vi "Histogram Plot save.vi"(6 "R Con H":dbl[][](array[numeric]), 7 "Date":string, 8 "error in":errorcluster caption="エラー入力", 9 "Normalized Plot Graph":dbl[][](graph), 10 "Plot Graph":dbl[][](graph), 11 "Folder Path":string) -> (0 "error out":errorcluster caption="エラー出力")   [LabVIEW 2018]
panel:
  out "Normalized Histogram":dbl[][](array[numeric])
  out "Count Historam":i32[][](array[numeric])
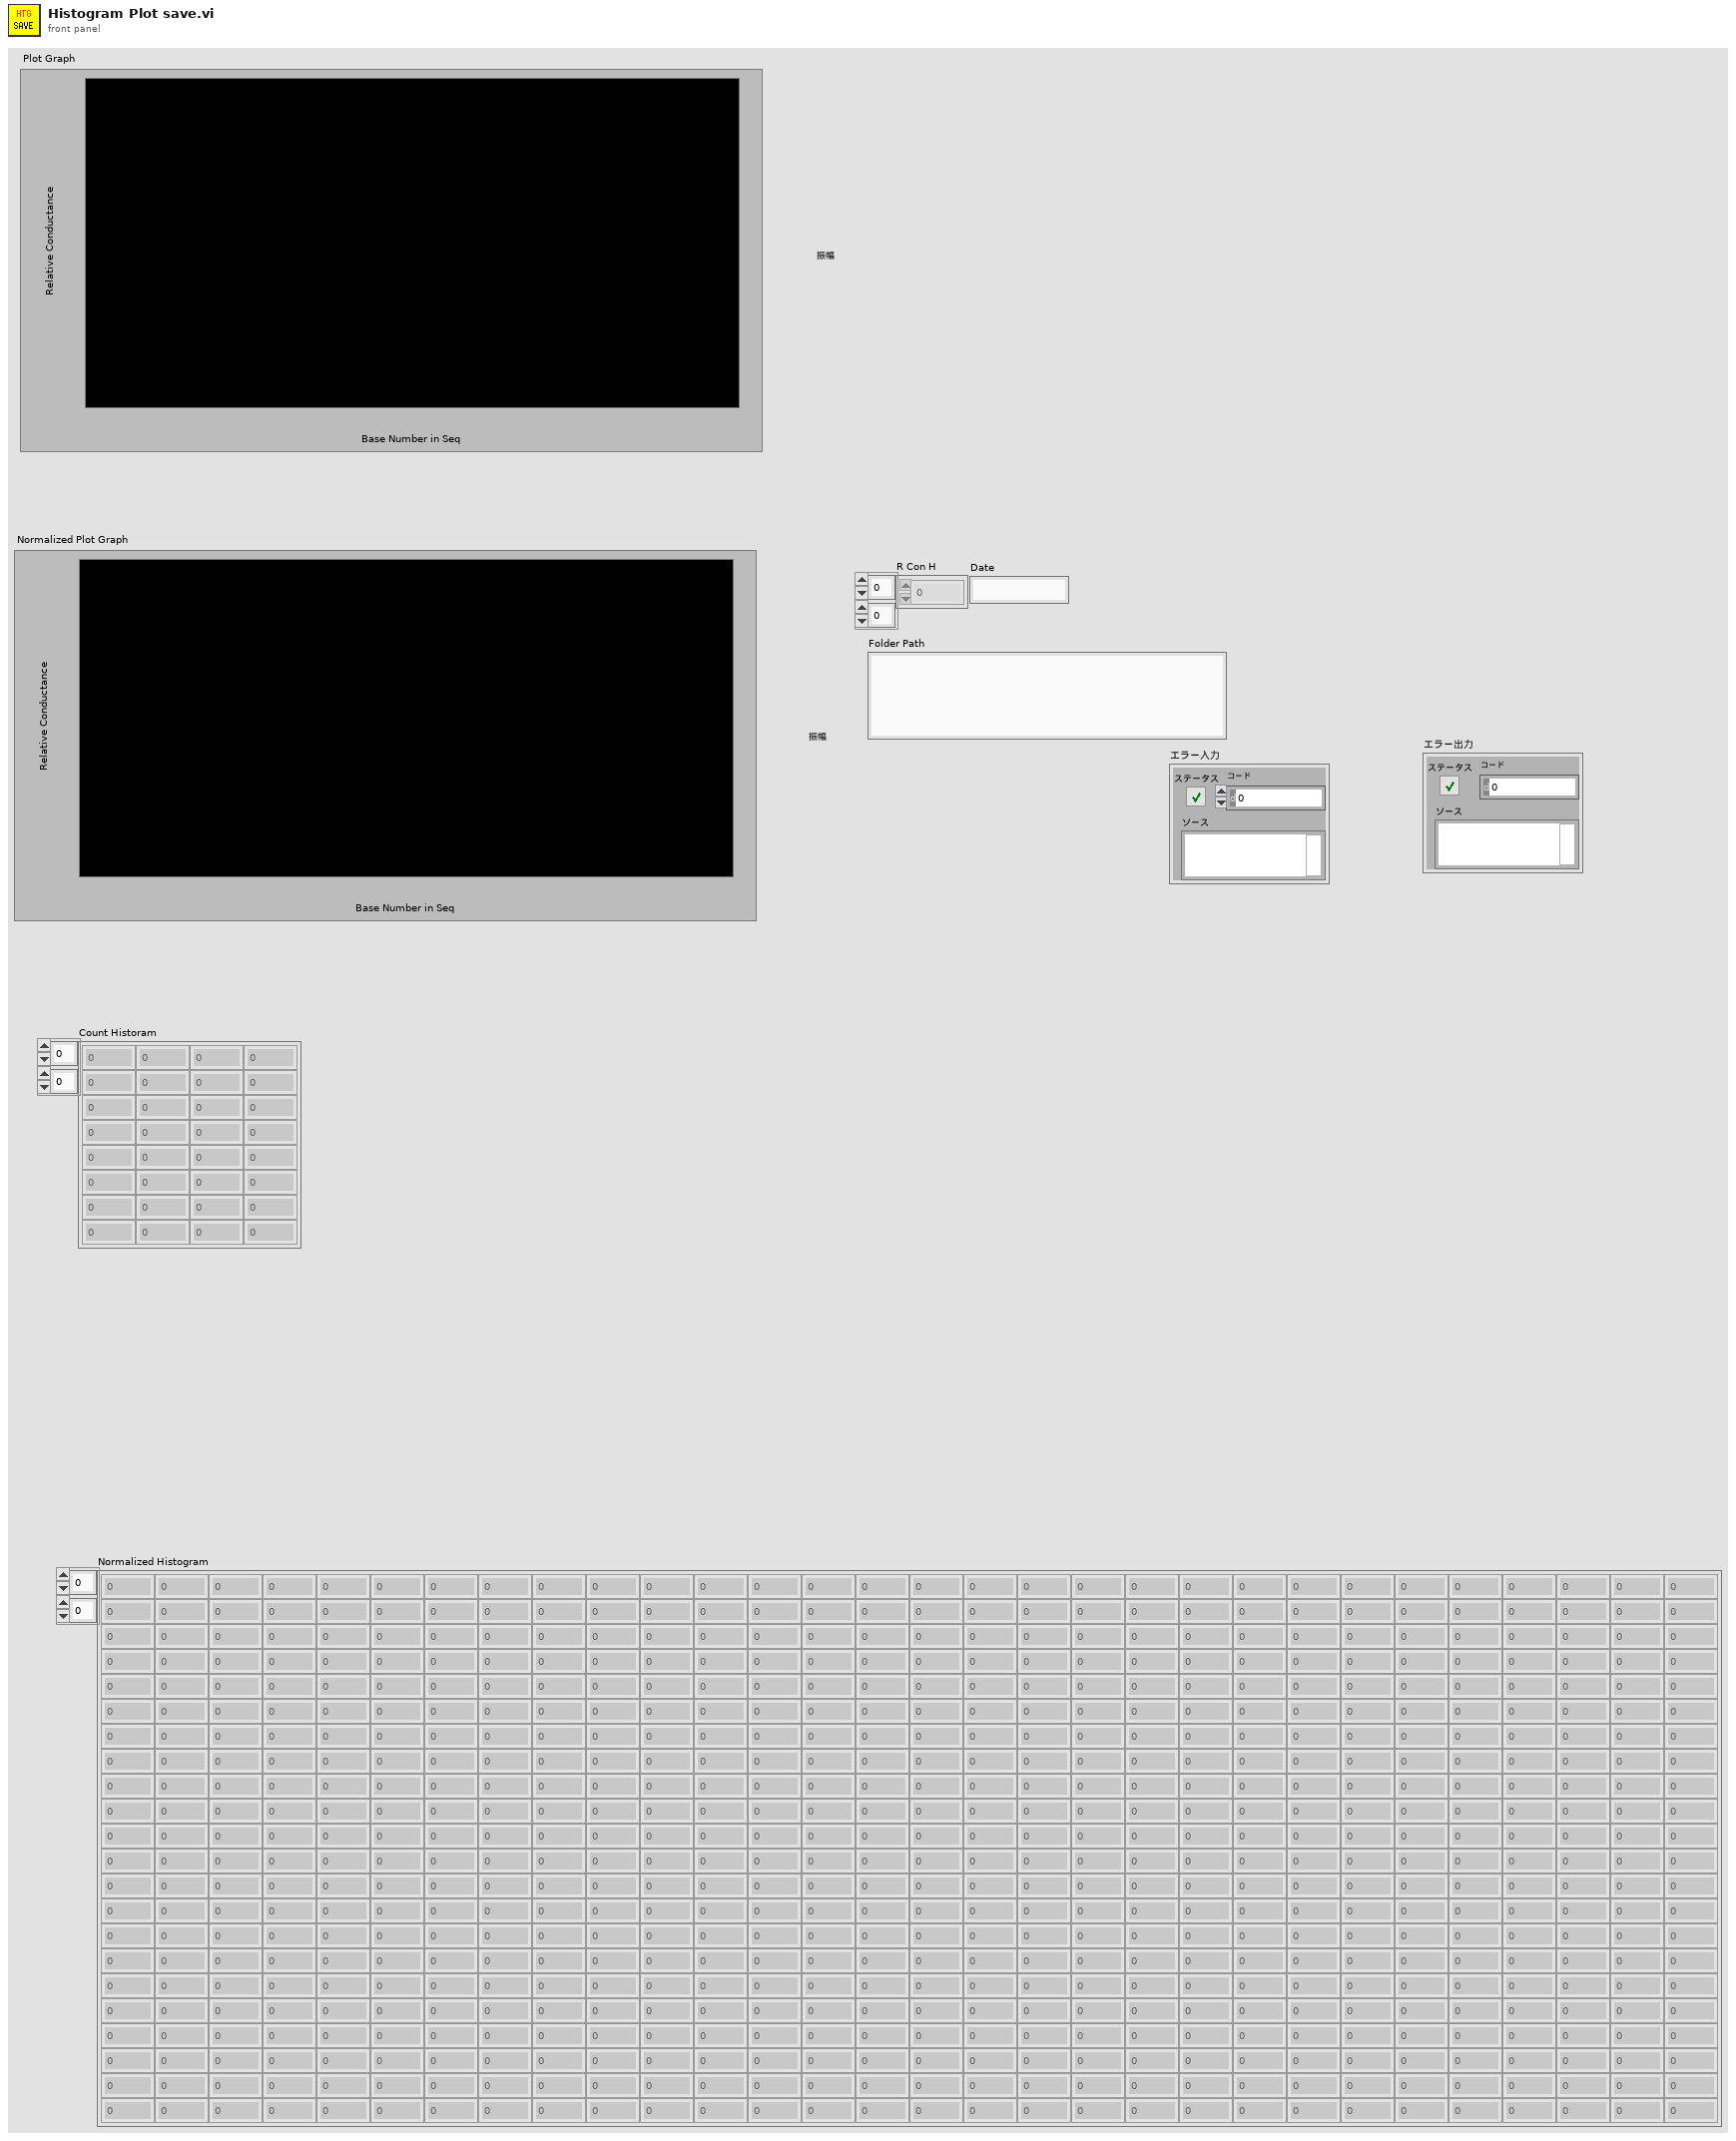
[diagram p1: front panel]
types:
  T1 = enum16{"open", "replace", "create", "open or create", "replace or create", "replace or create with confirmation"}
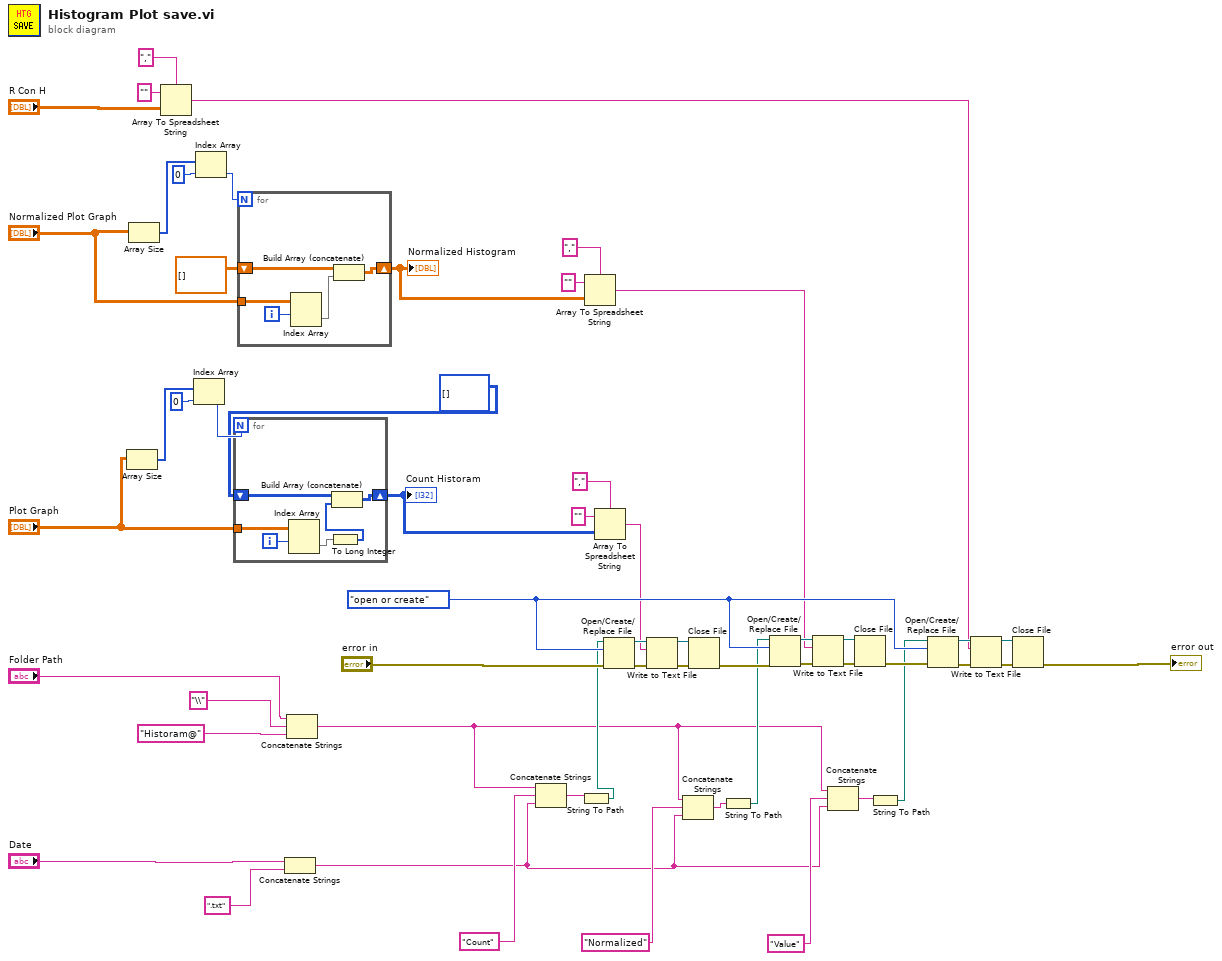
[diagram p0: block diagram]
diagram:
  w19 = T1."open or create" ("操作（0:open）")
  n1 = Array Size(array="Plot Graph") -> (size(s)=w54:i32[])
  n2 = Array Size(array="Normalized Plot Graph") -> (size(s)=w51:i32[])
  n3 = Array To Spreadsheet String(delimiter (Tab)="," ("デリミタ（タブ）"), array="R Con H", 3:"" ("形式文字列")) -> (spreadsheet string=w5:string)
  n4 = Index Array(array=w54, index=0 ("指標")) -> (element=w52:i32)
  n5 = Index Array(array=w51, index=0 ("指標")) -> (element=w49:i32)
  n6 = for {
    N: w52 -> [_]
    tunnel: "Plot Graph" -> [w61]
    shift-right: [w59] -> w44
    shift-left: i32[][] [] ("指標") -> [w58]
    i -> [w60]
    n7 = Index Array(array=w61, index (row)=w60) -> (element=w57:dbl[])  [unwired: 1 in]
    n8 = To Long Integer(number=w57) -> (32bit integer=w56:i32[])
    n9 = Build Array (concatenate)(w58, w56) -> (w59:i32[][])
  }
  "Count Historam" <- w44
  n10 = for {
    N: w49 -> [_]
    tunnel: "Normalized Plot Graph" -> [w66]
    shift-right: [w63] -> w39
    shift-left: dbl[][] [] -> [w62]
    i -> [w65]
    n11 = Index Array(array=w66, index (row)=w65) -> (element=w64:dbl[])  [unwired: 1 in]
    n12 = Build Array (concatenate)(w62, w64) -> (w63:dbl[][])
  }
  "Normalized Histogram" <- w39
  n13 = Concatenate Strings("Date", ".txt" ("文字列")) -> (w4:string)
  n14 = Concatenate Strings("Folder Path", "\\" ("文字列"), "Historam@" ("文字列")) -> (w3:string)
  n15 = Concatenate Strings(w3, "Count" ("文字列"), w4) -> (w13:string)
  n16 = String To Path(string=w13) -> (path=w12:path)
  n17 = Array To Spreadsheet String(delimiter (Tab)="," ("デリミタ（タブ）"), array=w39, 3:"" ("形式文字列")) -> (spreadsheet string=w6:string)
  n18 = Array To Spreadsheet String(delimiter (Tab)="," ("デリミタ（タブ）"), array=w44, 3:"" ("形式文字列")) -> (spreadsheet string=w7:string)
  n19 = Open/Create/Replace File(file path (use dialog)=w12, error in="error in", operation (0:open)=w19) -> (refnum out=w34:refnum<file>, error out=w35:errorcluster)  [unwired: 3 in, 1 out]
  n20 = Write to Text File(file (use dialog)=w34, text=w7, error in=w35) -> (refnum out=w33:refnum<file>, error out=w32:errorcluster)  [unwired: 1 in, 1 out]
  n21 = Concatenate Strings(w3, "Normalized" ("文字列"), w4) -> (w11:string)
  n22 = Close File(refnum=w33, error in=w32) -> (error out=w21:errorcluster)  [unwired: 1 out]
  n23 = String To Path(string=w11) -> (path=w10:path)
  n24 = Open/Create/Replace File(file path (use dialog)=w10, error in=w21, operation (0:open)=w19) -> (refnum out=w30:refnum<file>, error out=w31:errorcluster)  [unwired: 3 in, 1 out]
  n25 = Write to Text File(file (use dialog)=w30, text=w6, error in=w31) -> (refnum out=w29:refnum<file>, error out=w28:errorcluster)  [unwired: 1 in, 1 out]
  n26 = Concatenate Strings(w3, "Value" ("文字列"), w4) -> (w9:string)
  n27 = Close File(refnum=w29, error in=w28) -> (error out=w20:errorcluster)  [unwired: 1 out]
  n28 = String To Path(string=w9) -> (path=w8:path)
  n29 = Open/Create/Replace File(file path (use dialog)=w8, error in=w20, operation (0:open)=w19) -> (refnum out=w26:refnum<file>, error out=w27:errorcluster)  [unwired: 3 in, 1 out]
  n30 = Write to Text File(file (use dialog)=w26, text=w5, error in=w27) -> (refnum out=w25:refnum<file>, error out=w24:errorcluster)  [unwired: 1 in, 1 out]
  n31 = Close File(refnum=w25, error in=w24) -> (error out=→"error out":errorcluster)  [unwired: 1 out]
